vi "Get Statistics.vi"(6 "timeout (ms)":i32=5000, 8 "error in":errorcluster, 11 "gRPC ID":T2) -> (0 "error out":errorcluster, 2 "Statistics":T1, 3 "gRPC ID out":T2)   [LabVIEW 2021, in "CAN_Reader_CANsub_Wrapper.lvlib"]
uses:
  CAN_Reader_CANsub_Wrapper.lvlib
  <vilib>/gRPC/LabVIEW gRPC Library/Shared/grpcId.ctl
  CanReaderCansub_client/RPC Messages/cif_can_reader_cansub_Statistics.ctl
  CanReaderCansub_client/CanReaderCansub_client.lvlib
  <vilib>/gRPC/LabVIEW gRPC Library/grpc-lvsupport-release.lvlib
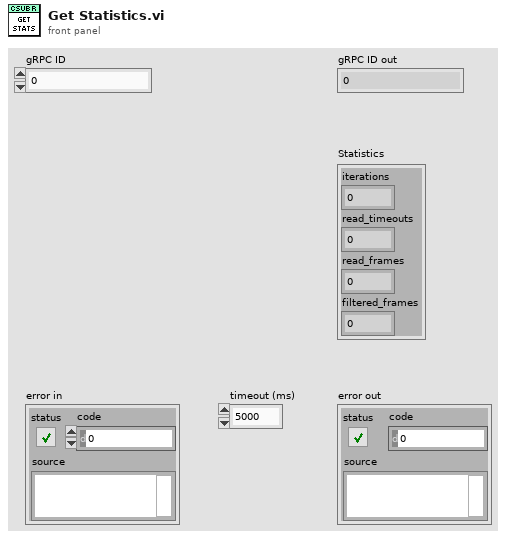
[diagram p1: front panel]
types:
  T1 = typedef "CanReaderCansub_client.lvlib/cif_can_reader_cansub_Statistics.ctl" = cluster{"iterations":u64, "read_timeouts":u64, "read_frames":u64, "filtered_frames":u64}
  T2 = typedef "grpc-lvsupport-release.lvlib/grpcId.ctl" = u64
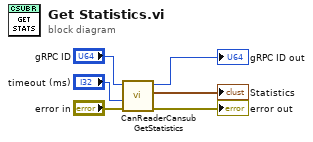
[diagram p0: block diagram]
diagram:
  n1 = call "CanReaderCansub GetStatistics.vi"("error in"="error in", "timeout (ms)"="timeout (ms)", "gRPC ID"="gRPC ID") -> ("error out"=→"error out":errorcluster, "Response Data"=→"Statistics":T1, "gRPC ID out"=→"gRPC ID out":T2)  [unwired: 6 in]
